vi "parse TDMS file.vi"(6 "Channel Types":T1[](array[typedef]), 8 "error in":errorcluster, 9 "channel name(s) in":string[](array[string]), 10 "group names in":string[](array[string]), 11 "file path":path) -> (0 "error out":errorcluster, 1 "channel names":string[](array[string]), 2 "group names":string[](array[string]), 3 "Array":dbl[][](array[numeric]), 5 "property values":string[](array[string]), 7 "property names":string[](array[string]))   [LabVIEW 2015, in "tdms logger tests.lvlib"]
uses:
  tdms logger tests.lvlib
  <vilib>/NI/Tag Bus/tag/Data Type.ctl
  <vilib>/NI/Tag Bus/tag/tag descriptor.lvclass
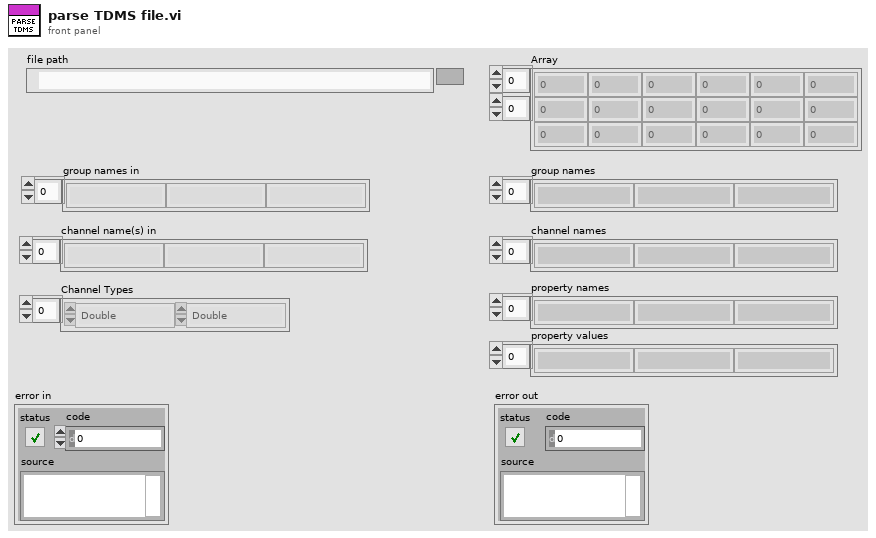
[diagram p1: front panel]
types:
  T1 = typedef "tag bus.lvlib/tag descriptor.lvclass/Data Type.ctl" = enum16{"Double", "Single", "I64", "I32", "I16", "I8", "U64", "U32", "U16", "U8", "Boolean", "String", "Array of Double", "Array of Single", "Array of I64", "Array of I32", "Array of I16", "Array of I8", "Array of U64", "Array of U32", "Array of U16", "Array of U8", "Array of Boolean", "Array of String"}
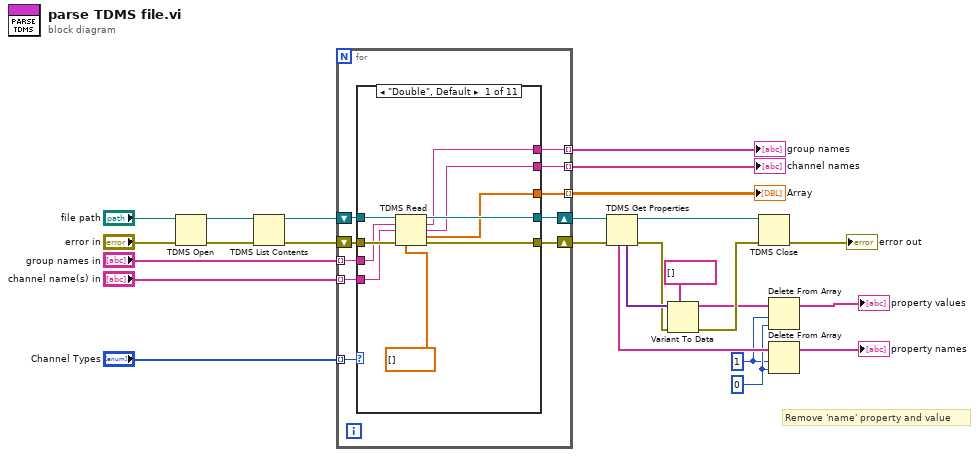
[diagram p0: block diagram]
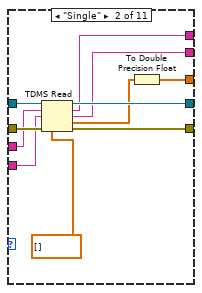
[diagram p2: hidden frame]
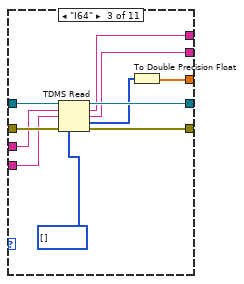
[diagram p3: hidden frame]
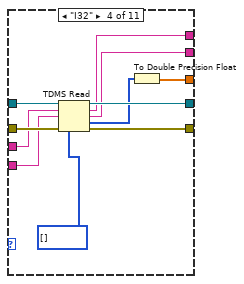
[diagram p4: hidden frame]
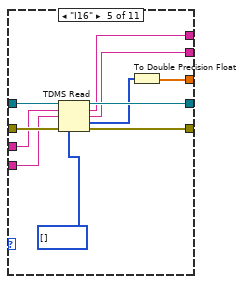
[diagram p5: hidden frame]
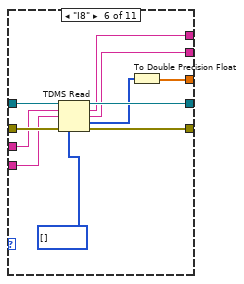
[diagram p6: hidden frame]
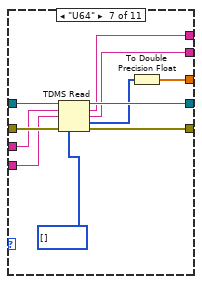
[diagram p7: hidden frame]
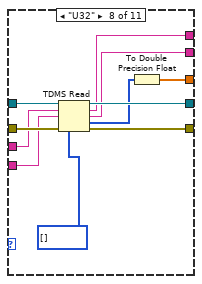
[diagram p8: hidden frame]
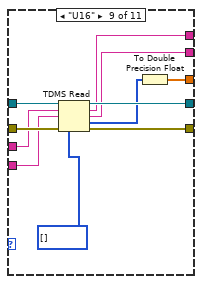
[diagram p9: hidden frame]
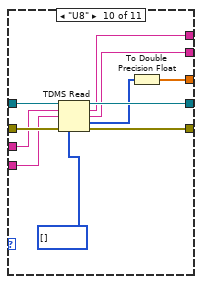
[diagram p10: hidden frame]
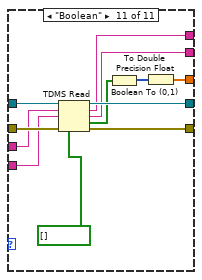
[diagram p11: hidden frame]
diagram:
  w6 = 0 ("length")
  w5 = 1 ("length")
  # "Remove 'name' property and value"
  n1 = TDMS Open(8:"error in", 11:"file path") -> (0:w24:errorcluster, 3:w25:refnum<k34>)  [unwired: 5 in]
  n2 = TDMS List Contents(4:w24, 7:w25) -> (0:w22:errorcluster, 3:w23:refnum<k34>)  [unwired: 1 in, 2 out]
  n3 = for {
    tunnel: "group names in" -> [w30] mode=indexing
    tunnel: "channel name(s) in" -> [w29] mode=indexing
    shift-right: [w27] -> w15
    shift-left: w22 -> [w35]
    shift-right: [w34] -> w17
    shift-left: w23 -> [w33]
    tunnel: "Channel Types" -> [w36] mode=indexing
    tunnel: [w32] -> w3 mode=indexing
    tunnel: [w31] -> w2 mode=indexing
    tunnel: [w28] -> w1 mode=indexing
    n4 = case shown="\"Double\", Default" w36 {
      tunnel: w35 -> [w46 w56 w67 w78 w89 w100 w111 w122 w133 w144 w156]
      tunnel: [w43 w54 w66 w77 w88 w99 w110 w121 w132 w143 w155] -> w27
      tunnel: [w44 w53 w65 w76 w87 w98 w109 w120 w131 w142 w154] -> w34
      tunnel: w33 -> [w45 w55 w64 w75 w86 w97 w108 w119 w130 w141 w153]
      tunnel: [w41 w51 w63 w74 w85 w96 w107 w118 w129 w140 w152] -> w32
      tunnel: [w40 w52 w62 w73 w84 w95 w106 w117 w128 w139 w151] -> w31
      tunnel: w30 -> [w38 w48 w61 w72 w83 w94 w105 w116 w127 w138 w150]
      tunnel: w29 -> [w37 w47 w60 w71 w82 w93 w104 w115 w126 w137 w149]
      tunnel: [w39 w49 w58 w69 w80 w91 w102 w113 w124 w135 w146] -> w28
      frame "Double", Default {
        n5 = TDMS Read(0:w45, 5:w38, 7:w37, 11:w46, 12:dbl[] []) -> (4:w44:refnum<k34>, 6:w41:string, 8:w40:string, 10:w39:dbl[], 15:w43:errorcluster)  [unwired: 3 in, 1 out]
      }
      frame "Single" {
        n6 = TDMS Read(0:w55, 5:w48, 7:w47, 11:w56, 12:sgl[] []) -> (4:w53:refnum<k34>, 6:w51:string, 8:w52:string, 10:w50:sgl[], 15:w54:errorcluster)  [unwired: 3 in, 1 out]
        n7 = To Double Precision Float(number=w50) -> (double precision float=w49:dbl[])
      }
      frame "I64" {
        n8 = TDMS Read(0:w64, 5:w61, 7:w60, 11:w67, 12:i64[] []) -> (4:w65:refnum<k34>, 6:w63:string, 8:w62:string, 10:w59:i64[], 15:w66:errorcluster)  [unwired: 3 in, 1 out]
        n9 = To Double Precision Float(number=w59) -> (double precision float=w58:dbl[])
      }
      frame "I32" {
        n10 = TDMS Read(0:w75, 5:w72, 7:w71, 11:w78, 12:i32[] []) -> (4:w76:refnum<k34>, 6:w74:string, 8:w73:string, 10:w70:i32[], 15:w77:errorcluster)  [unwired: 3 in, 1 out]
        n11 = To Double Precision Float(number=w70) -> (double precision float=w69:dbl[])
      }
      frame "I16" {
        n12 = TDMS Read(0:w86, 5:w83, 7:w82, 11:w89, 12:i16[] []) -> (4:w87:refnum<k34>, 6:w85:string, 8:w84:string, 10:w81:i16[], 15:w88:errorcluster)  [unwired: 3 in, 1 out]
        n13 = To Double Precision Float(number=w81) -> (double precision float=w80:dbl[])
      }
      frame "I8" {
        n14 = TDMS Read(0:w97, 5:w94, 7:w93, 11:w100, 12:i8[] []) -> (4:w98:refnum<k34>, 6:w96:string, 8:w95:string, 10:w92:i8[], 15:w99:errorcluster)  [unwired: 3 in, 1 out]
        n15 = To Double Precision Float(number=w92) -> (double precision float=w91:dbl[])
      }
      frame "U64" {
        n16 = TDMS Read(0:w108, 5:w105, 7:w104, 11:w111, 12:u64[] []) -> (4:w109:refnum<k34>, 6:w107:string, 8:w106:string, 10:w103:u64[], 15:w110:errorcluster)  [unwired: 3 in, 1 out]
        n17 = To Double Precision Float(number=w103) -> (double precision float=w102:dbl[])
      }
      frame "U32" {
        n18 = TDMS Read(0:w119, 5:w116, 7:w115, 11:w122, 12:u32[] []) -> (4:w120:refnum<k34>, 6:w118:string, 8:w117:string, 10:w114:u32[], 15:w121:errorcluster)  [unwired: 3 in, 1 out]
        n19 = To Double Precision Float(number=w114) -> (double precision float=w113:dbl[])
      }
      frame "U16" {
        n20 = TDMS Read(0:w130, 5:w127, 7:w126, 11:w133, 12:u16[] []) -> (4:w131:refnum<k34>, 6:w129:string, 8:w128:string, 10:w125:u16[], 15:w132:errorcluster)  [unwired: 3 in, 1 out]
        n21 = To Double Precision Float(number=w125) -> (double precision float=w124:dbl[])
      }
      frame "U8" {
        n22 = TDMS Read(0:w141, 5:w138, 7:w137, 11:w144, 12:u8[] []) -> (4:w142:refnum<k34>, 6:w140:string, 8:w139:string, 10:w136:u8[], 15:w143:errorcluster)  [unwired: 3 in, 1 out]
        n23 = To Double Precision Float(number=w136) -> (double precision float=w135:dbl[])
      }
      frame "Boolean" {
        n24 = TDMS Read(0:w153, 5:w150, 7:w149, 11:w156, 12:bool[] []) -> (4:w154:refnum<k34>, 6:w152:string, 8:w151:string, 10:w148:bool[], 15:w155:errorcluster)  [unwired: 3 in, 1 out]
        n25 = Boolean To (0,1)(Boolean=w148) -> (0, 1=w147:i16[])
        n26 = To Double Precision Float(number=w147) -> (double precision float=w146:dbl[])
      }
    }
  }
  "group names" <- w3
  "Array" <- w1
  "channel names" <- w2
  n27 = TDMS Get Properties(8:w15, 11:w17) -> (0:w12:errorcluster, 3:w16:refnum<k34>, 4:w14:variant[], 6:w8:string[])  [unwired: 4 in, 2 out]
  n28 = Variant To Data(error in=w12, type=string[] [] ("property values"), Variant=w14) -> (data=w10:string[], error out=w11:errorcluster)
  n29 = TDMS Close(8:w11, 11:w16) -> (0:→"error out":errorcluster)  [unwired: 1 out]
  n30 = Delete From Array(array=w10, length=w5, index=w6) -> (array with subset deleted=→"property values":string[])  [unwired: 1 out]
  n31 = Delete From Array(array=w8, length=w5, index=w6) -> (array with subset deleted=→"property names":string[])  [unwired: 1 out]
